vi "Run TCS.vi"(8 "error in (no error)":errorcluster, 11 "SPARC4_GEI in":refnum<class "S4GEI.lvclass">) -> (0 "error out":errorcluster, 3 "SPARC4_GEI out":refnum<class "S4GEI.lvclass">)   [LabVIEW 2018, in "S4GEI.lvclass"]
uses:
  S4GEI.lvclass
  TCS/TCS.lvclass
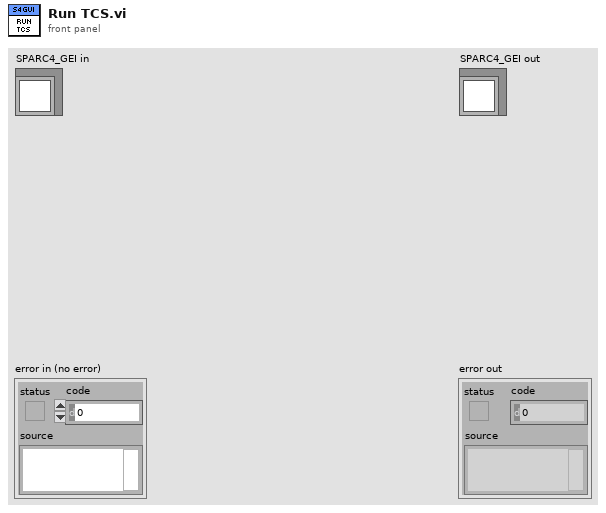
[diagram p1: front panel]
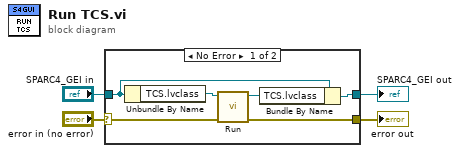
[diagram p0: block diagram]
diagram:
  n1 = case shown="No Error" "error in (no error)" {
    selector: "error in (no error)" -> [w5 w12]
    tunnel: [w9 w12] -> w3
    tunnel: [w10 w11] -> w2
    tunnel: "SPARC4_GEI in" -> [w8 w11]
    frame No Error {
      n2 = Unbundle By Name(w8) -> ("TCS.lvclass"=w6:refnum<class "TCS.lvclass">)
      n3 = call "Run.vi"("error in (no error)"=w5, "TCS in"=w6) -> ("error out"=w9:errorcluster, "TCS out"=w7:refnum<class "TCS.lvclass">)  [unwired: 8 in]
      n4 = Bundle By Name(cluster=w8, "TCS.lvclass"=w7) -> (w10:refnum<class "S4GEI.lvclass">)
    }
    frame Error {
    }
  }
  "error out" <- w3
  "SPARC4_GEI out" <- w2
